vi "VIH Project - Control Rule - Merge Rule Arrays.vi"(10 "Control Rules":T1[](array[typedef]), 11 "Parent Control Rules":T1[](array[typedef])) -> (2 "Control Rules out":T1[](array[typedef]))   [LabVIEW 2014]
doc: "::: VI Helpeks :::\nCopyright (c) 2000-2026 Konstantin Shifershteyn. All rights reserved."
uses:
  _VIH HelpGen.llb/VIH HelpGen Typedef - Cluster - Control Rule.ctl
  _VIH HelpGen.llb/VIH HelpGen Typedef - Enum - Description Mode.ctl
  _VIH HelpGen.llb/VIH HelpGen Typedef - Enum - Default,Enable,Disable.ctl
  _VIH HelpGen.llb/VIH HelpGen Typedef - Cluster - Enum Value Info.ctl
panel:
  # "VI Helpeks\nCopyright (c) 2012-2026 Konstantin Shifershteyn"
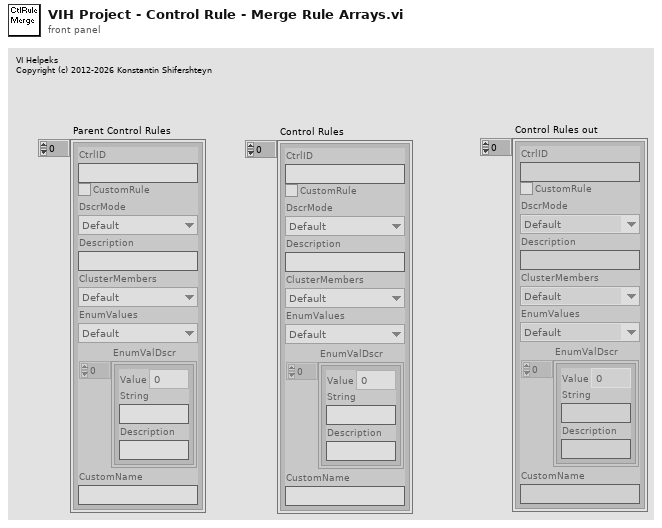
[diagram p1: front panel]
types:
  T1 = typedef "VIH HelpGen Typedef - Cluster - Control Rule.ctl" = cluster{"CtrlID":string, "CustomRule":bool, "DscrMode":T2, "Description":string, "ClusterMembers":T3, "EnumValues":T3, "EnumValDscr":T4[], "CustomName":string}
  T2 = typedef "VIH HelpGen Typedef - Enum - Description Mode.ctl" = enum16{"Default", "Description", "Description1", "Description2", "Custom", "None"}
  T3 = typedef "VIH HelpGen Typedef - Enum - Default,Enable,Disable.ctl" = enum16{"Default", "Enable", "Disable"}
  T4 = typedef "VIH HelpGen Typedef - Cluster - Enum Value Info.ctl" = cluster{"Value":ext, "String":string, "Description":string}
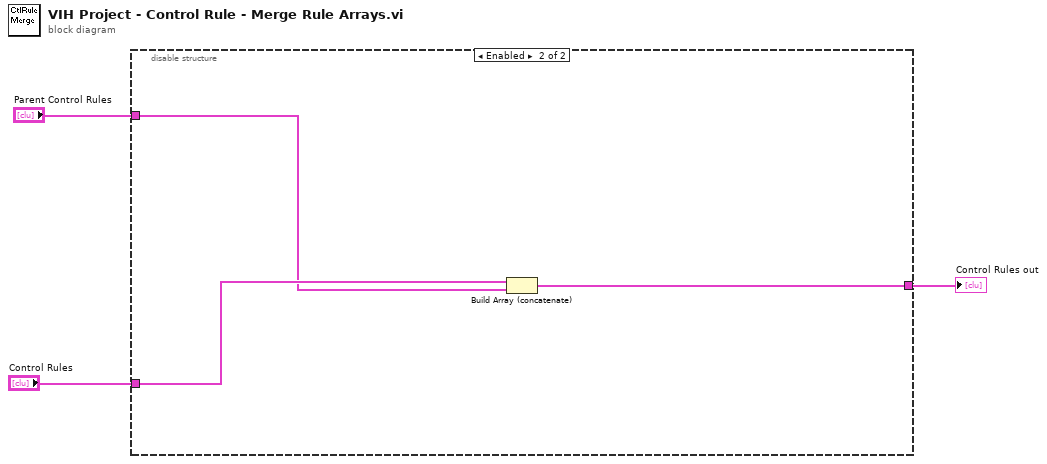
[diagram p0: block diagram]
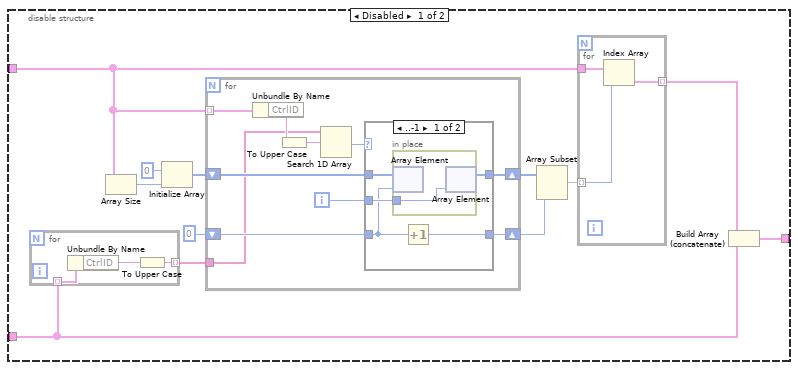
[diagram p2: hidden frame]
diagram:
  n1 = disable-structure shown="Enabled" {
    disable-tunnel: "Parent Control Rules" -> [w8 w41]
    disable-tunnel: "Control Rules" -> [w5 w42]
    disable-tunnel: [w4 w40] -> w1
    frame Disabled {
      n2 = for {
        tunnel: w5 -> [w18] mode=indexing
        tunnel: [w16] -> w7 mode=indexing
        n3 = Unbundle By Name(w18) -> ("CtrlID"=w17:string)
        n4 = To Upper Case(1:w17) -> (0:w16:string)
      }
      n5 = Array Size(array=w8) -> (size(s)=w15:i32)
      n6 = Initialize Array(0, w15) -> (w13:i32[])
      n7 = for {
        tunnel: w8 -> [w31] mode=indexing
        shift-right: [w28] -> w11
        shift-left: w13 -> [w30]
        shift-right: [w26] -> w10
        shift-left: 0 -> [w27]
        tunnel: w7 -> [w22]
        i -> [w29]
        n8 = Unbundle By Name(w31) -> ("CtrlID"=w24:string)
        n9 = To Upper Case(1:w24) -> (0:w25:string)
        n10 = Search 1D Array(1D array=w22, element=w25) -> (index of element=w23:i32)  [unwired: 1 in]
        n11 = case shown="..-1" w23 {
          tunnel: w30 -> [w36 w39]
          tunnel: w29 -> [w35 _]
          tunnel: [w34 w39] -> w28
          tunnel: w27 -> [w33 w38]
          tunnel: [w32 w38] -> w26
          frame ..-1 {
            n12 = in-place {
              in-place-border: w35 -> [w37]
              n13 = in-place-array #1(w36, w33) -> ()  [unwired: 1 out]
              n14 = in-place-array #1(w37) -> (w34:i32[])  [unwired: 1 out]
            }
            n15 = Increment(x=w33) -> (x+1=w32:i32)
          }
          frame 0.. {
          }
        }
      }
      n16 = Array Subset(array=w11, length=w10) -> (w9:i32[])  [unwired: 1 in]
      n17 = for {
        tunnel: w8 -> [w21]
        tunnel: w9 -> [w20] mode=indexing
        tunnel: [w19] -> w6 mode=indexing
        n18 = Index Array(array=w21, index=w20) -> (element=w19:T1)
      }
      n19 = Build Array (concatenate)(w6, w5) -> (w4:T1[])
    }
    frame Enabled {
      n20 = Build Array (concatenate)(w42, w41) -> (w40:T1[])
    }
  }
  "Control Rules out" <- w1
